vi "Write-Read data.vi"(8 "error in":errorcluster, 9 "data string in":string, 10 "JSON string in":string, 11 "connection ID":refnum<k5>) -> (0 "error out":errorcluster, 1 "data string out":string, 2 "JSON string out":string, 3 "connection ID out":refnum<k5>)   [LabVIEW 2020, in "LabVIEW-Python TCP Lib.lvlib"]
uses:
  LabVIEW-Python TCP Lib.lvlib
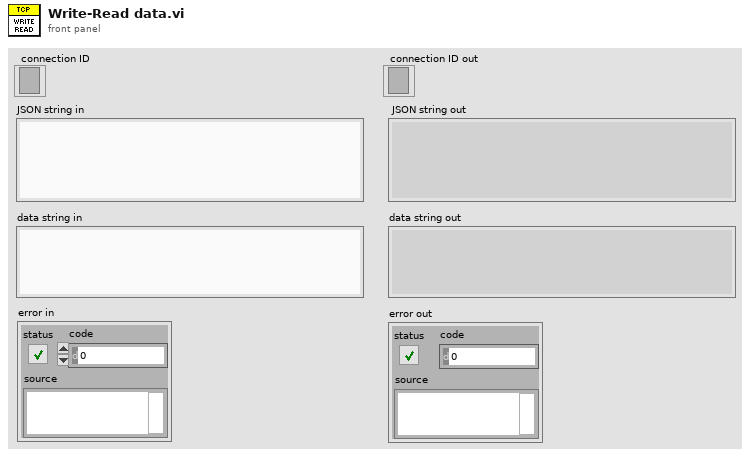
[diagram p1: front panel]
types:
  T1 = enum16{"big-endian, network order", "native, host order", "little-endian"}
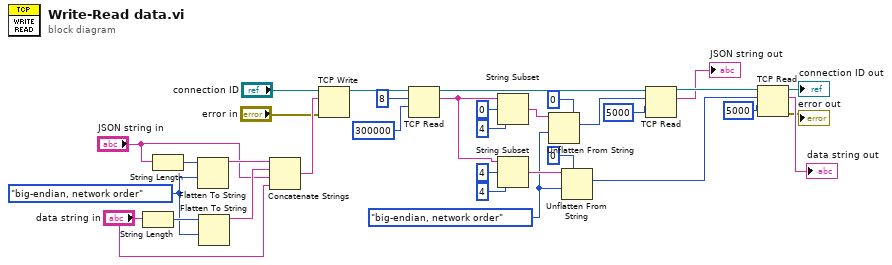
[diagram p0: block diagram]
diagram:
  w16 = T1."big-endian, network order" ("byte order (0:big-endian, network order)")
  w5 = T1."big-endian, network order" ("byte order (0:big-endian, network order)")
  n1 = String Length(string="data string in") -> (length=w31:i32)
  n2 = String Length(string="JSON string in") -> (length=w32:i32)
  n3 = Flatten To String(anything=w32, byte order (0:big-endian, network order)=w5) -> (data string=w33:string)  [unwired: 2 in, 2 out]
  n4 = Flatten To String(anything=w31, byte order (0:big-endian, network order)=w5) -> (data string=w30:string)  [unwired: 2 in, 2 out]
  n5 = Concatenate Strings(w33, w30, "JSON string in", "data string in") -> (w8:string)
  n6 = TCP Write(connection ID="connection ID", data in=w8, error in (no error)="error in") -> (connection ID out=w26:refnum<k5>)  [unwired: 1 in, 2 out]
  n7 = TCP Read(connection ID=w26, bytes to read=8, 9:300000 ("timeout ms (25000)")) -> (connection ID out=w14:refnum<k5>, data out=w21:string)  [unwired: 2 in, 1 out]
  n8 = String Subset(string=w21, offset (0)=0, length (rest)=4 ("length (rest)")) -> (substring=w20:string)
  n9 = String Subset(string=w21, offset (0)=4, length (rest)=4 ("length (rest)")) -> (substring=w18:string)
  n10 = Unflatten From String(type=0 ("offset (0)"), binary string=w20, byte order (0:big-endian, network order)=w16) -> (value=w13:i32)  [unwired: 2 in, 2 out]
  n11 = Unflatten From String(type=0 ("offset (0)"), binary string=w18, byte order (0:big-endian, network order)=w16) -> (value=w10:i32)  [unwired: 2 in, 2 out]
  n12 = TCP Read(connection ID=w14, bytes to read=w13, 9:5000 ("timeout ms (25000)")) -> (connection ID out=w11:refnum<k5>, data out=→"JSON string out":string)  [unwired: 2 in, 1 out]
  n13 = TCP Read(connection ID=w11, bytes to read=w10, 9:5000 ("timeout ms (25000)")) -> (connection ID out=→"connection ID out":refnum<k5>, data out=→"data string out":string, error out=→"error out":errorcluster)  [unwired: 2 in]
